vi "Dispose.vi"(8 "error in (no error)":errorcluster, 11 "View in":refnum<class "View.lvclass">) -> (0 "error out":errorcluster, 3 "View out":refnum<class "View.lvclass">)   [LabVIEW 2024, in "View.lvclass"]
uses:
  View.lvclass
  View.lvclass/View.ctl
  Viewmodel/Viewmodel.lvclass
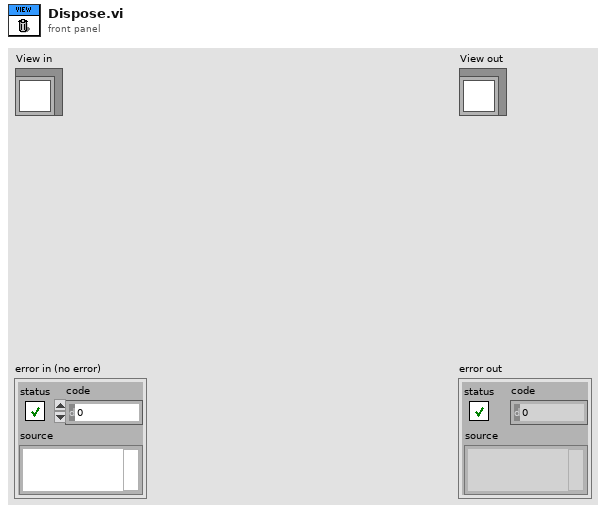
[diagram p1: front panel]
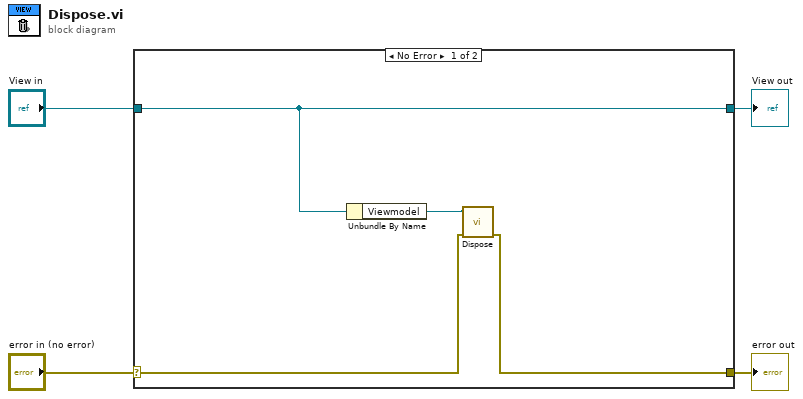
[diagram p0: block diagram]
diagram:
  n1 = case shown="No Error" "error in (no error)" {
    selector: "error in (no error)" -> [w6 w10]
    tunnel: [w5 w10] -> w3
    tunnel: [w8 w9] -> w1
    tunnel: "View in" -> [w8 w9]
    frame No Error {
      n2 = Unbundle By Name(w8) -> ("Viewmodel"=w7:refnum<class "Viewmodel.lvclass">)
      n3 = call-dynamic "Dispose.vi"("error in (no error)"=w6, "ChangeNotifier in"=w7) -> ("error out"=w5:errorcluster)  [unwired: 8 in, 1 out]
    }
    frame Error {
    }
  }
  "error out" <- w3
  "View out" <- w1
